vi "Wait for Iteration Notification.vi"(8 "error in (no error)":errorcluster, 10 "timeout in ms (-1)":i32, 11 "Iterator NR Actor in":refnum<class "Iterator NR Actor.lvclass">) -> (0 "error out":errorcluster, 1 "timed out?":bool, 2 "Iterate?":bool, 3 "Iterator NR Actor out":refnum<class "Iterator NR Actor.lvclass">)   [LabVIEW 2023, in "Iterator Actor.lvlib" / "Iterator NR Actor.lvclass"]
uses:
  Iterator NR Actor.lvclass
  Iterator NR Actor.lvclass/Iterator NR Actor.ctl
  <userlib>/_OpenG.lib/error/error.llb/openg_error.lvlib
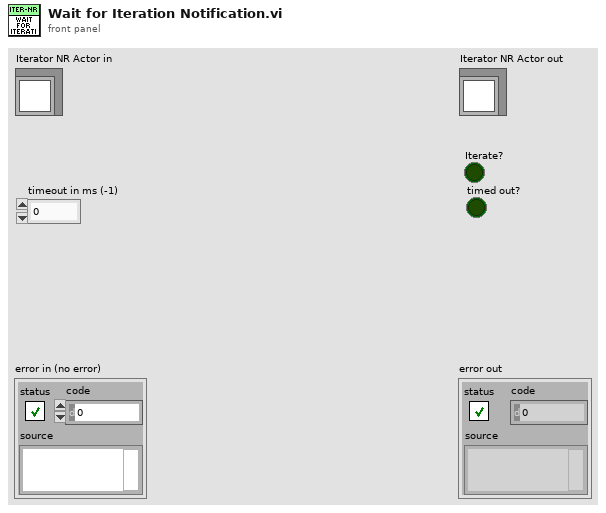
[diagram p1: front panel]
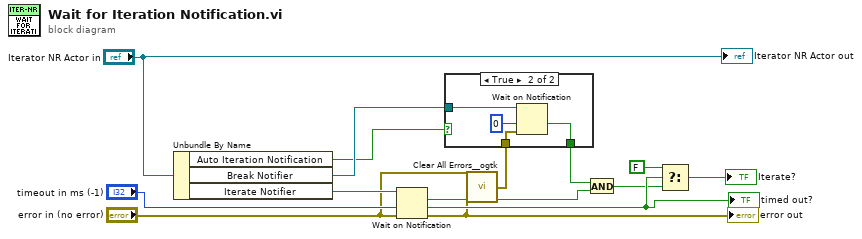
[diagram p0: block diagram]
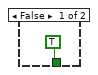
[diagram p2: hidden frame]
diagram:
  n1 = Unbundle By Name("Iterator NR Actor in") -> ("Auto Iteration Notification"=w7:bool, "Break Notifier"=w8:refnum<notifier>, "Iterate Notifier"=w13:refnum<notifier>)
  n2 = Wait on Notification(notifier=w13, timeout in ms (-1)="timeout in ms (-1)", error in (no error)="error in (no error)") -> (notification=w5:bool, timed out?=w11:bool, error out=w3:errorcluster)  [unwired: 1 in, 1 out]
  "error out" <- w3
  "timed out?" <- w11
  n3 = call <userlib>:"Clear All Errors__ogtk.vi"("Upsteam Error (optional)"="error in (no error)", "Error In"=w3) -> ("Error Out"=w2:errorcluster)  [unwired: 2 in]
  n4 = case shown="True" w7 {
    tunnel: w2 -> [_ w19]
    tunnel: w8 -> [_ w18]
    tunnel: [TRUE ("timed out?") w16] -> w6
    frame False {
    }
    frame True {
      n5 = Wait on Notification(notifier=w18, timeout in ms (-1)=0, error in (no error)=w19) -> (timed out?=w16:bool)  [unwired: 1 in, 3 out]
    }
  }
  n6 = And(x=w6, y=w5) -> (x .and. y?=w4:bool)
  n7 = Select(t=FALSE, s=w11, f=w4) -> (s? t:f=→"Iterate?":bool)
  "Iterator NR Actor out" <- "Iterator NR Actor in"
